vi "C-885 Device Engine.vi"(0 "Unique Notifier Name":string, 11 "Axis Names":string[](array[string])) -> ()   [LabVIEW 2016]
uses:
  Stages Controls/Stage Notifier Element.ctl
  Stages Controls/Stage Actions.ctl
  Stages Controls/Stage Status.ctl
  C-885 Type Defs/C-885 Chassis Status.ctl
panel:
  in  "Halt":bool
  in  "Velocity":dbl
  in  "Get Pos":bool
  out "Var Error":bool
  in  "Quit":bool
  in  "Init Axes":bool
  in  "Axes Positions":dbl[](array[numeric])
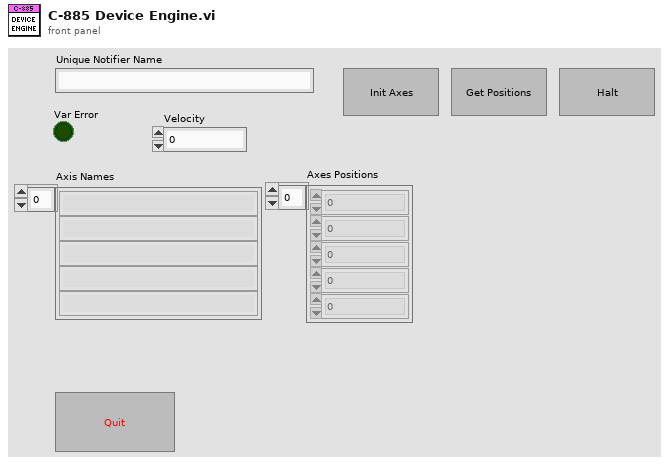
[diagram p1: front panel]
types:
  T1 = typedef "C-885 Chassis Status.ctl" = enum16{"Avalible", "Busy", "Halt"}
  T2 = typedef "Stage Notifier Element.ctl" = cluster{"Action":T3, "Axis":bool[], "Setpoint":dbl[], "Velocity":dbl, "Cmd Recvd?":bool, "Position":dbl[], "Status":T4, "Misc":variant}
  T3 = typedef "Stage Actions.ctl" = enum16{"Get Position", "MVR", "MOVE", "HALT", "ONTARGET", "ERROR", "REFERENCE", "INIT", "VELOCITY", "STATUS", "EXIT", "HOME", "ZEROPOS", "NANOPOS", "ANALOG", "QUIT"}
  T4 = typedef "Stage Status.ctl" = enum16{"Error", "Abort", "Busy", "On Target"}
  T5 = enum32{"Invalid", "Standard", "Closed", "Hidden", "Minimized", "Maximized"}
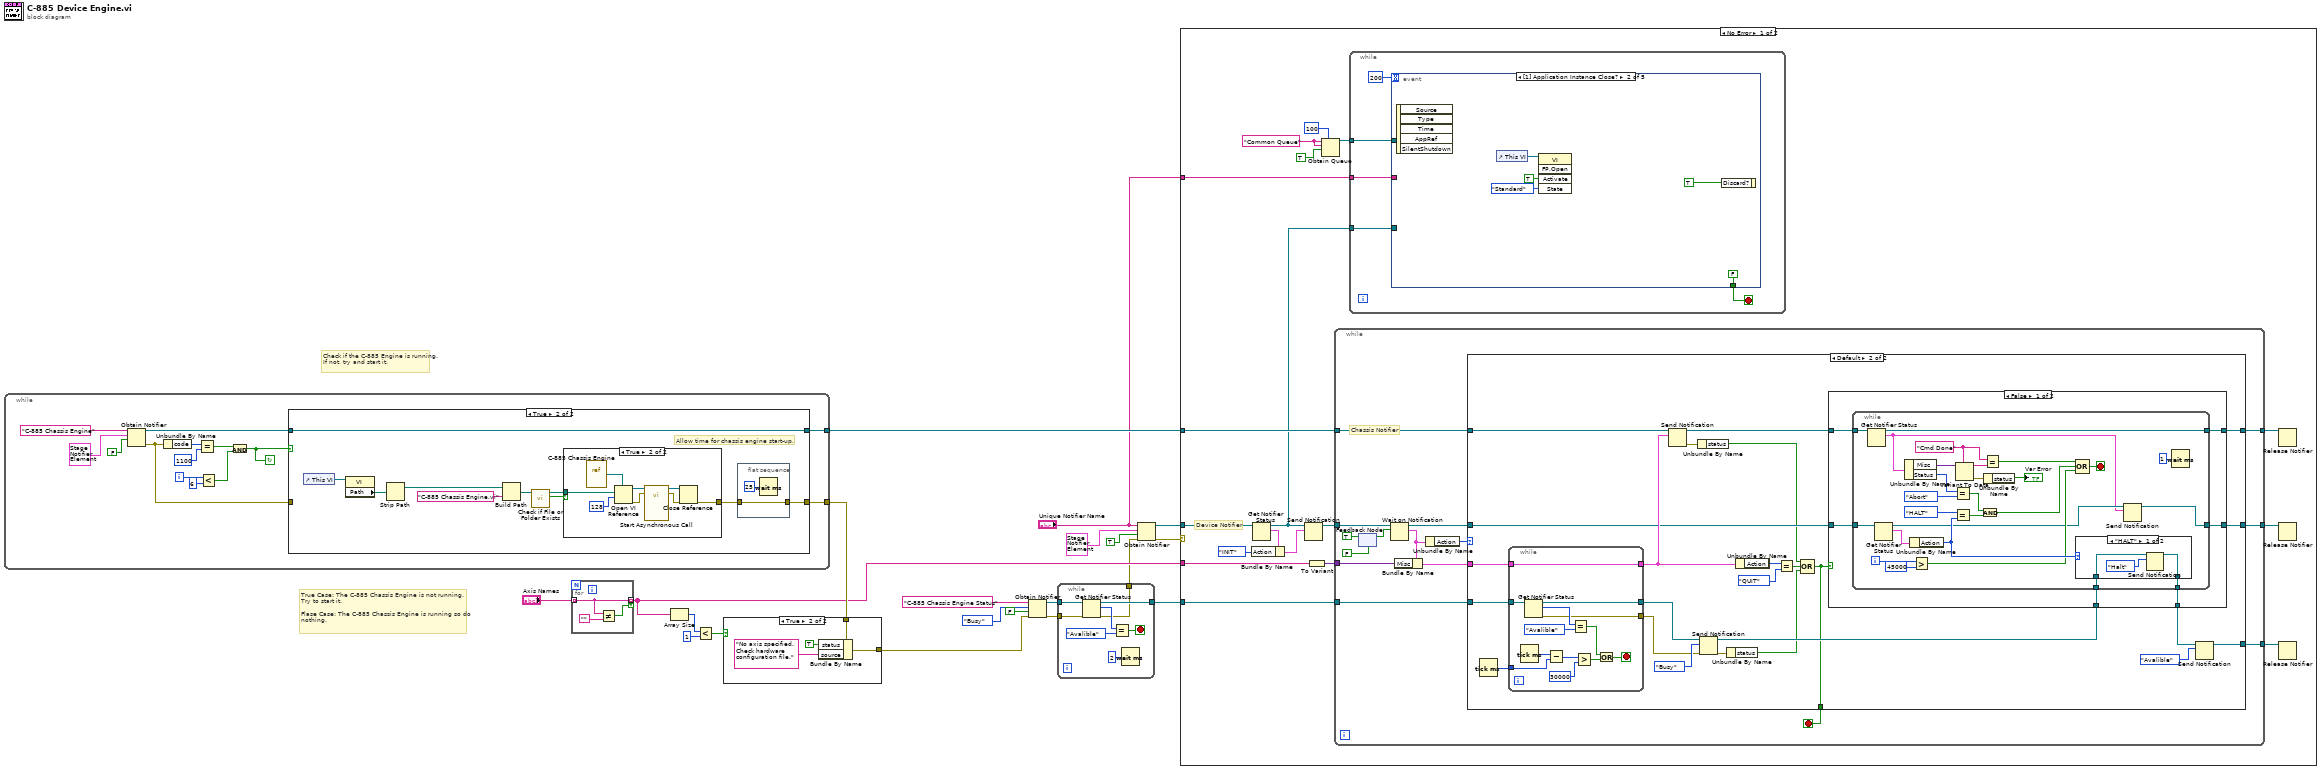
[diagram p0: block diagram]
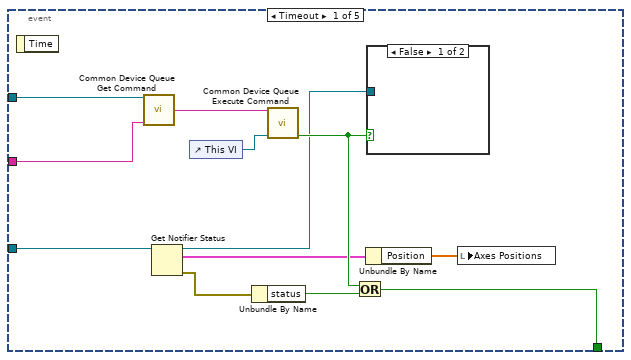
[diagram p2: hidden frame]
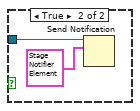
[diagram p3: hidden frame]
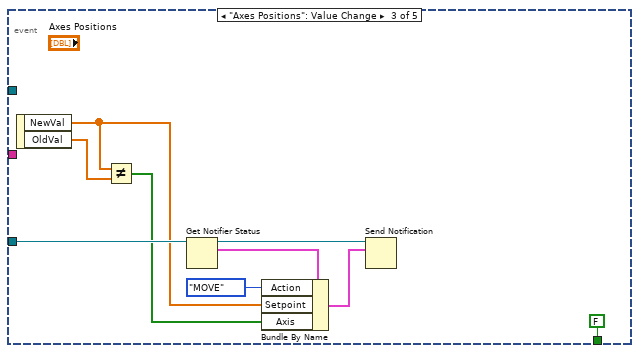
[diagram p4: hidden frame]
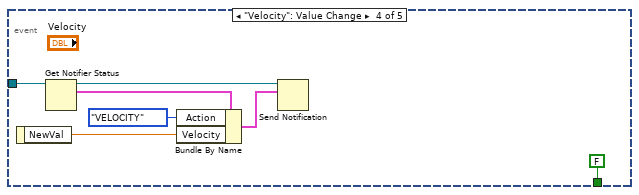
[diagram p5: hidden frame]
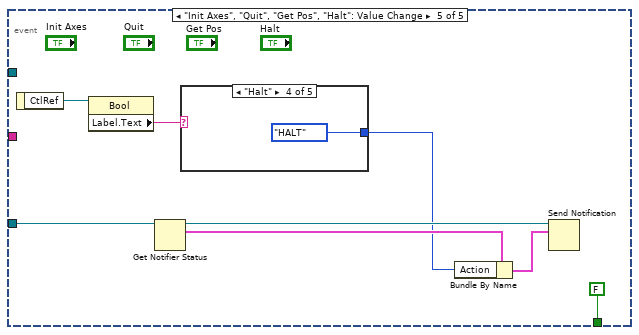
[diagram p6: hidden frame]
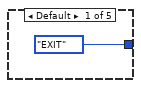
[diagram p7: hidden frame]
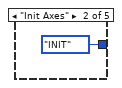
[diagram p8: hidden frame]
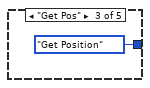
[diagram p9: hidden frame]
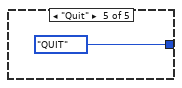
[diagram p10: hidden frame]
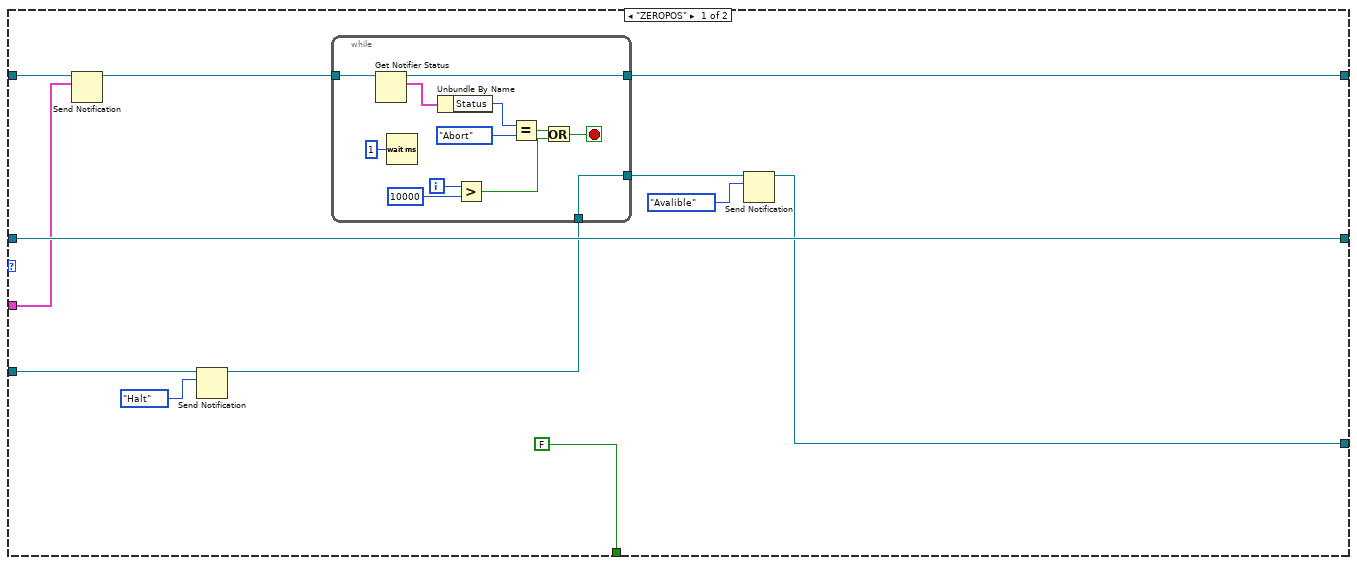
[diagram p11: hidden frame]
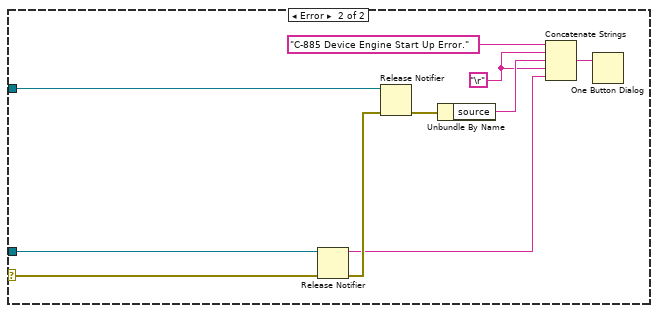
[diagram p14: hidden frame]
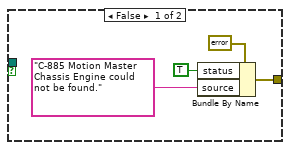
[diagram p17: hidden frame]
diagram:
  # "Check if the C-885 Engine is running. If not, try and start it."
  # "True Case: The C-885 Chassis Engine is not running.\nTry to start it.\n\nFlase Case: The C-885 Chassis Engine is running so do\nnothing."
  n1 = while {
    tunnel: [w28] -> w14
    tunnel: [w23] -> w7
    i -> [w30]
    stop <- w25 continue-if-true
    n2 = Obtain Notifier(name (unnamed)="C-885 Chassis Engine", notification data type=T2 {"Action"=enum."Get Position", "Axis"=[], "Setpoint"=[], "Velocity"=0.5, "Cmd Recvd?"=FALSE, "Position"=[], "Status"=enum."Error", "Misc"=variant} ("Stage Status"), create if not found? (T)=FALSE) -> (notifier out=w34:refnum<notifier>, error out=w22:errorcluster)  [unwired: 1 in, 1 out]
    n3 = Unbundle By Name(w22) -> ("code"=w33:i32)
    n4 = Equal?(x=w33, y=1100) -> (x = y?=w26:bool)
    n5 = Less?(x=w30, y=6) -> (x < y?=w27:bool)
    n6 = And(x=w26, y=w27) -> (x .and. y?=w25:bool)
    n7 = case shown="True" w25 {
      tunnel: w34 -> [w36 w46]
      tunnel: [w36 w46] -> w28
      tunnel: [w35 w37] -> w23
      tunnel: w22 -> [w35 _]
      frame False {
      }
      frame True {
        # "Allow time for chassis engine start-up."
        n8 = control-ref of="This VI"() -> (w41:refnum<vi>)
        n9 = property class="VI"(reference=w41) -> ("Path"=w42:path)  [unwired: 1 in, 2 out]
        n10 = Strip Path(path=w42) -> (stripped path=w43:path)  [unwired: 1 out]
        n11 = Build Path(base path=w43, name or relative path="C-885 Chassis Engine.vi" ("name (unnamed)")) -> (appended path=w45:path)
        n12 = call <vilib>:"Check if File or Folder Exists.vi"("path"=w45) -> ("file or folder exists?"=w40:bool, "dup path"=w39:path)  [unwired: 8 in, 1 out]
        n13 = case shown="True" w40 {
          tunnel: w39 -> [_ w54]
          tunnel: [w49 w53] -> w38
          frame False {
            n14 = Bundle By Name(cluster=errorcluster {"status"=FALSE, "code"=0, "source"=""} ("Error"), "status"=TRUE, "source"="C-885 Motion Master Chassis Engine could not be found.") -> (w49:errorcluster)
          }
          frame True {
            n15 = vi-ref "C-885 Chassis Engine.vi"() -> (w59:refnum<vi>)
            n16 = Open VI Reference(type specifier VI Refnum (for type only)=w59, vi path=w54, options=128) -> (vi reference=w58:refnum<vi>, error out=w56:errorcluster)  [unwired: 3 in]
            n17 = call-by-ref "Start Asynchronous Call"(reference=w58, error in=w56) -> (reference out=w57:refnum<vi>, error out=w55:errorcluster)  [unwired: 16 in]
            n18 = Close Reference(reference=w57, error in (no error)=w55) -> (error out=w53:errorcluster)
          }
        }
        n19 = flat-sequence {
          tunnel: w38 -> [w48]
          tunnel: [w48] -> w37
          frame #0 {
            n20 = Wait (ms)(milliseconds to wait=u32 25) -> ()  [unwired: 1 out]
          }
        }
      }
    }
  }
  n21 = for {
    tunnel: "Axis Names" -> [w62] mode=indexing
    tunnel: [w62] -> w6 mode=indexing if=w61
    n22 = Not Equal?(x=w62, y="") -> (x != y?=w61:bool)
  }
  n23 = Array Size(array=w6) -> (size(s)=w18:i32)
  n24 = Less?(x=w18, y=1) -> (x < y?=w16:bool)
  n25 = case shown="True" w16 {
    tunnel: w7 -> [w64 w68]
    tunnel: [w64 w65] -> w3
    frame False {
    }
    frame True {
      n26 = Bundle By Name(cluster=w68, "status"=TRUE, "source"="No axis specified. Check hardware configuration file.") -> (w65:errorcluster)
    }
  }
  n27 = Obtain Notifier(name (unnamed)="C-885 Chassis Engine Status", notification data type=C-885_Chassis_Status."Busy" ("C-885 Status"), create if not found? (T)=FALSE, error in (no error)=w3) -> (notifier out=w11:refnum<notifier>, error out=w4:errorcluster)  [unwired: 1 out]
  n28 = while {
    tunnel: w11 -> [w76]
    tunnel: [w73] -> w5
    tunnel: [w70] -> w2
    tunnel: w4 -> [w69]
    stop <- w72 stop-if-true
    n29 = Get Notifier Status(notifier=w76, error in (no error)=w69) -> (notifier out=w73:refnum<notifier>, current notification=w74:T1, error out=w70:errorcluster)  [unwired: 2 out]
    n30 = Equal?(x=w74, y=C-885_Chassis_Status."Avalible") -> (x = y?=w72:bool)
    n31 = Wait (ms)(milliseconds to wait=u32 2) -> ()  [unwired: 1 out]
  }
  n32 = Obtain Notifier(name (unnamed)="Unique Notifier Name", notification data type=T2 {"Action"=enum."INIT", "Axis"=[], "Setpoint"=[], "Velocity"=0.5, "Cmd Recvd?"=FALSE, "Position"=[], "Status"=enum."Error", "Misc"=variant} ("Stage Status"), create if not found? (T)=TRUE, error in (no error)=w2) -> (notifier out=w15:refnum<notifier>, error out=w1:errorcluster)  [unwired: 1 out]
  n33 = case shown="No Error" w1 {
    selector: w1 -> [_ w271]
    tunnel: w15 -> [w82 w273]
    tunnel: w14 -> [w90 w272]
    tunnel: w6 -> [w94 _]
    tunnel: "Unique Notifier Name" -> [w84 _]
    tunnel: w5 -> [w77 _]
    frame No Error {
      w88 = "Common Queue" ("Unique Notifier Name")
      # "Device Notifier"
      n34 = Get Notifier Status(notifier=w82) -> (notifier out=w78:refnum<notifier>, current notification=w81:T2)  [unwired: 1 in, 3 out]
      n35 = Bundle By Name(cluster=w81, "Action"=Stage_Actions."INIT") -> (w79:T2)
      n36 = Send Notification(notification=w79, notifier=w78) -> (notifier out=w83:refnum<notifier>)  [unwired: 1 in, 1 out]
      n37 = To Variant(anything=w94) -> (Variant=w93:variant)
      n38 = Obtain Queue(max queue size (-1, unlimited)=100, name (unnamed)=w88, element data type=w88, create if not found? (T)=TRUE) -> (queue out=w85:refnum<queue>)  [unwired: 1 in, 2 out]
      n39 = while {
        tunnel: w90 -> [w161]
        tunnel: w83 -> [w162]
        tunnel: w93 -> [w160]
        tunnel: [w157] -> w91
        tunnel: [w158] -> w92
        tunnel: w77 -> [w156]
        tunnel: [w153] -> w89
        stop <- w159 stop-if-true
        # "Chassis Notifier"
        n40 = feedback-in #1(TRUE ("ignore previous (F)")) -> ()
        n41 = feedback #1(FALSE) -> (w149:bool)
        n42 = Wait on Notification(notifier=w162, ignore previous (F)=w149) -> (notifier out=w154:refnum<notifier>, notification=w152:T2)  [unwired: 2 in, 2 out]
        n43 = Bundle By Name(cluster=w152, "Misc"=w160) -> (w155:T2)
        n44 = Unbundle By Name(w152) -> ("Action"=w151:T3)
        n45 = case shown="Default" w151 {
          tunnel: w161 -> [w165 w210]
          tunnel: [FALSE w188] -> w159
          tunnel: [w170 w206] -> w158
          tunnel: [w171 w205] -> w157
          tunnel: w156 -> [w172 w204]
          tunnel: w155 -> [w163 w203]
          tunnel: w154 -> [w171 w199]
          tunnel: [w166 w194] -> w153
          frame "ZEROPOS" {
            n46 = Send Notification(notification=w163, notifier=w165) -> (notifier out=w164:refnum<notifier>)  [unwired: 1 in, 1 out]
            n47 = Send Notification(notification=C-885_Chassis_Status."Halt", notifier=w172) -> (notifier out=w169:refnum<notifier>)  [unwired: 1 in, 1 out]
            n48 = while {
              tunnel: w164 -> [w186]
              tunnel: [w185] -> w170
              tunnel: w169 -> [w175]
              tunnel: [w175] -> w167
              i -> [w180]
              stop <- w176 stop-if-true
              n49 = Get Notifier Status(notifier=w186) -> (notifier out=w185:refnum<notifier>, current notification=w184:T2)  [unwired: 1 in, 3 out]
              n50 = Wait (ms)(milliseconds to wait=u32 1) -> ()  [unwired: 1 out]
              n51 = Unbundle By Name(w184) -> ("Status"=w183:T4)
              n52 = Greater?(x=w180, y=10000) -> (0:w177:bool)
              n53 = Equal?(x=w183, y=Stage_Status."Abort") -> (x = y?=w178:bool)
              n54 = Or(x=w178, y=w177) -> (x .or. y?=w176:bool)
            }
            n55 = Send Notification(notification=C-885_Chassis_Status."Avalible", notifier=w167) -> (notifier out=w166:refnum<notifier>)  [unwired: 1 in, 1 out]
          }
          frame Default {
            n56 = Tick Count (ms)() -> (millisecond timer value=w187:u32)
            n57 = while {
              tunnel: w204 -> [w263]
              tunnel: [w260] -> w201
              tunnel: [w259] -> w202
              tunnel: w203 -> [w259]
              tunnel: [w258] -> w193
              tunnel: w187 -> [w256]
              stop <- w251 stop-if-true
              n58 = Tick Count (ms)() -> (millisecond timer value=w257:u32)
              n59 = Get Notifier Status(notifier=w263) -> (notifier out=w260:refnum<notifier>, current notification=w262:T1, error out=w258:errorcluster)  [unwired: 1 in, 2 out]
              n60 = Subtract(x=w257, y=w256) -> (x-y=w255:u32)
              n61 = Equal?(x=w262, y=C-885_Chassis_Status."Avalible") -> (x = y?=w252:bool)
              n62 = Greater?(x=w255, y=u32 30000) -> (0:w253:bool)
              n63 = Or(x=w252, y=w253) -> (x .or. y?=w251:bool)
            }
            n64 = Send Notification(notification=w202, notifier=w210) -> (notifier out=w207:refnum<notifier>, error out=w198:errorcluster)  [unwired: 1 in]
            n65 = Unbundle By Name(w198) -> ("status"=w190:bool)
            n66 = Send Notification(notification=C-885_Chassis_Status."Busy", notifier=w201, error in (no error)=w193) -> (notifier out=w196:refnum<notifier>, error out=w192:errorcluster)
            n67 = Unbundle By Name(w192) -> ("status"=w189:bool)
            n68 = Unbundle By Name(w202) -> ("Action"=w209:T3)
            n69 = Equal?(x=w209, y=Stage_Actions."QUIT") -> (x = y?=w191:bool)
            n70 = Compound Arithmetic op=OR(w190, w191, w189) -> (w188:bool)
            n71 = case shown="False" w188 {
              tunnel: w207 -> [w216 w250]
              tunnel: [w215 w250] -> w206
              tunnel: [w214 w249] -> w205
              tunnel: w199 -> [w213 w249]
              tunnel: w196 -> [w212 w248]
              tunnel: [w211 w248] -> w195
              frame False {
                n72 = while {
                  tunnel: w216 -> [w243]
                  tunnel: w213 -> [w241]
                  tunnel: [w242] -> w215
                  tunnel: [w218] -> w214
                  tunnel: w212 -> [w238]
                  tunnel: [w237] -> w211
                  i -> [w232]
                  stop <- w236 stop-if-true
                  w228 = "Cmd Done"
                  n73 = Get Notifier Status(notifier=w243) -> (notifier out=w242:refnum<notifier>, current notification=w217:T2)  [unwired: 1 in, 3 out]
                  n74 = Get Notifier Status(notifier=w241) -> (notifier out=w219:refnum<notifier>, current notification=w239:T2)  [unwired: 1 in, 3 out]
                  n75 = Unbundle By Name(w217) -> ("Misc"=w234:variant, "Status"=w224:T4)
                  n76 = Unbundle By Name(w239) -> ("Action"=w235:T3)
                  n77 = Greater?(x=w232, y=45000) -> (0:w230:bool)
                  n78 = Equal?(x=w224, y=Stage_Status."Abort") -> (x = y?=w222:bool)
                  n79 = Equal?(x=Stage_Actions."HALT", y=w235) -> (x = y?=w221:bool)
                  n80 = Variant To Data(type=w228, Variant=w234) -> (data=w229:string, error out=w227:errorcluster)  [unwired: 1 in]
                  n81 = And(x=w222, y=w221) -> (x .and. y?=w220:bool)
                  n82 = Equal?(x=w228, y=w229) -> (x = y?=w233:bool)
                  n83 = Unbundle By Name(w227) -> ("status"=→"Var Error":bool)
                  n84 = case shown="\"HALT\"" w235 {
                    tunnel: w238 -> [w246 w247]
                    tunnel: [w245 w247] -> w237
                    frame "HALT" {
                      n85 = Send Notification(notification=C-885_Chassis_Status."Halt", notifier=w246) -> (notifier out=w245:refnum<notifier>)  [unwired: 1 in, 1 out]
                    }
                    frame Default {
                    }
                  }
                  n86 = Compound Arithmetic op=OR(w233, w220, w230) -> (w236:bool)
                  n87 = Send Notification(notification=w217, notifier=w219) -> (notifier out=w218:refnum<notifier>)  [unwired: 1 in, 1 out]
                  n88 = Wait (ms)(milliseconds to wait=u32 1) -> ()  [unwired: 1 out]
                }
              }
              frame True {
              }
            }
            n89 = Send Notification(notification=C-885_Chassis_Status."Avalible", notifier=w195) -> (notifier out=w194:refnum<notifier>)  [unwired: 1 in, 1 out]
          }
        }
      }
      n90 = while {
        tunnel: w78 -> [w96]
        tunnel: w85 -> [w98]
        tunnel: w84 -> [w97]
        stop <- w95 stop-if-true
        n91 = event shown="[1] Application Instance Close?" {
          selector: _ -> [_ _ _ _ _]
          dyn-events: _ -> [_ _ _ _ _]
          timeout: 200 -> [_ _ _ _ _]
          tunnel: w98 -> [w111 _ _ _ _]
          tunnel: w97 -> [w110 _ _ _ _]
          tunnel: w96 -> [w108 _ w126 w133 w139]
          tunnel: [w109 FALSE ("Boolean") FALSE FALSE ("Boolean") FALSE] -> w95
          event Timeout {
            n92 = event-data() -> ()  [unwired: 1 in, 1 out]
            n93 = call "Common Device Queue Get Command.vi"("Common Queue"=w111, "Notifier Name"=w110) -> ("Command"=w106:string)  [unwired: 12 in, 1 out]
            n94 = Get Notifier Status(notifier=w108) -> (notifier out=w104:refnum<notifier>, current notification=w101:T2, error out=w103:errorcluster)  [unwired: 1 in, 2 out]
            n95 = control-ref of="This VI"() -> (w107:refnum<vi>)
            n96 = Unbundle By Name(w103) -> ("status"=w102:bool)
            n97 = call "Common Device Queue Execute Command.vi"("Common Command"=w106, "VI Refnum"=w107) -> ("Quit?"=w105:bool)  [unwired: 12 in, 1 out]
            n98 = Or(x=w105, y=w102) -> (x .or. y?=w109:bool)
            n99 = Unbundle By Name(w101) -> ("Position"=w100:dbl[])
            n100 = case shown="False" w105 {
              tunnel: w104 -> [_ w113]
              frame False {
              }
              frame True {
                n101 = Send Notification(notification=T2 {"Action"=enum."QUIT", "Axis"=[], "Setpoint"=[], "Velocity"=0.5, "Cmd Recvd?"=FALSE, "Position"=[], "Status"=enum."Error", "Misc"=variant} ("Stage Status"), notifier=w113) -> ()  [unwired: 1 in, 2 out]
              }
            }
            n102 = local write "Axes Positions"(w100) -> ()
          }
          event Application Instance Close? {
            n103 = event-data() -> ()  [unwired: 1 in, 5 out]
            n104 = control-ref of="This VI"() -> (w114:refnum<vi>)
            n105 = invoke class="VI" method="FP.Open"(reference=w114, "Activate"=TRUE ("Activate?"), "State"=T5."Standard") -> ()  [unwired: 2 in, 5 out]
            n106 = event-data("Discard?"=TRUE ("SilentShutdown")) -> ()  [unwired: 1 in, 1 out]
          }
          event "Axes Positions": Value Change {
            n107 = event-data() -> ("NewVal"=w120:dbl[], "OldVal"=w121:dbl[])  [unwired: 1 in]
            n108 = Not Equal?(x=w120, y=w121) -> (x != y?=w119:bool[])
            n109 = Get Notifier Status(notifier=w126) -> (notifier out=w123:refnum<notifier>, current notification=w125:T2)  [unwired: 1 in, 3 out]
            n110 = Bundle By Name(cluster=w125, "Action"=Stage_Actions."MOVE", "Setpoint"=w120, "Axis"=w119) -> (w122:T2)
            n111 = Send Notification(notification=w122, notifier=w123) -> ()  [unwired: 1 in, 2 out]
          }
          event "Velocity": Value Change {
            n112 = event-data() -> ("NewVal"=w128:dbl)  [unwired: 1 in]
            n113 = Get Notifier Status(notifier=w133) -> (notifier out=w132:refnum<notifier>, current notification=w131:T2)  [unwired: 1 in, 3 out]
            n114 = Bundle By Name(cluster=w131, "Action"=Stage_Actions."VELOCITY", "Velocity"=w128) -> (w130:T2)
            n115 = Send Notification(notification=w130, notifier=w132) -> ()  [unwired: 1 in, 2 out]
          }
          event "Init Axes", "Quit", "Get Pos", "Halt": Value Change {
            n116 = event-data() -> ("CtlRef"=w141:refnum<vi>)  [unwired: 1 in]
            n117 = property class="Bool"(reference=w141) -> ("Label.Text"=w140:string)  [unwired: 1 in, 2 out]
            n118 = Get Notifier Status(notifier=w139) -> (notifier out=w138:refnum<notifier>, current notification=w137:T2)  [unwired: 1 in, 3 out]
            n119 = case shown="\"Halt\"" w140 {
              tunnel: [Stage_Actions."EXIT" ("Action") Stage_Actions."INIT" ("Action") Stage_Actions."Get Position" ("Action") Stage_Actions."HALT" ("Action") Stage_Actions."QUIT" ("Action")] -> w135
              frame Default {
              }
              frame "Init Axes" {
              }
              frame "Get Pos" {
              }
              frame "Halt" {
              }
              frame "Quit" {
              }
            }
            n120 = Bundle By Name(cluster=w137, "Action"=w135) -> (w136:T2)
            n121 = Send Notification(notification=w136, notifier=w138) -> ()  [unwired: 1 in, 2 out]
          }
        }
      }
      n122 = Release Notifier(notifier=w92) -> ()  [unwired: 2 in, 3 out]
      n123 = Release Notifier(notifier=w91) -> ()  [unwired: 2 in, 3 out]
      n124 = Release Notifier(notifier=w89) -> ()  [unwired: 2 in, 3 out]
    }
    frame Error {
      w265 = "\r"
      n125 = Release Notifier(notifier=w273, error in (no error)=w271) -> (notifier name=w264:string, error out=w270:errorcluster)  [unwired: 1 in, 1 out]
      n126 = Release Notifier(notifier=w272, error in (no error)=w270) -> (error out=w266:errorcluster)  [unwired: 1 in, 2 out]
      n127 = Unbundle By Name(w266) -> ("source"=w268:string)
      n128 = Concatenate Strings("C-885 Device Engine Start Up Error.", w265, w268, w265, w264) -> (w267:string)
      n129 = One Button Dialog(message=w267) -> ()  [unwired: 1 in, 1 out]
    }
  }
